vi "VELOCIDAD.vi"() -> ()   [LabVIEW 2023]
uses:
  <vilib>/Instr/_visa.llb/Select Event Type.ctl
  <vilib>/Instr/_visa.llb/VISA Configure Serial Port (Instr).vi
panel:
  out "Waveform Graph":dbl[](graph)
  out "Array":dbl[](array[numeric])
  in  "stop":bool
  in  "setpoint 2":dbl=1000.0
  in  "enviar":bool
  out "read buffer":string
  in  "Puerto":refnum<visa-resource-name>
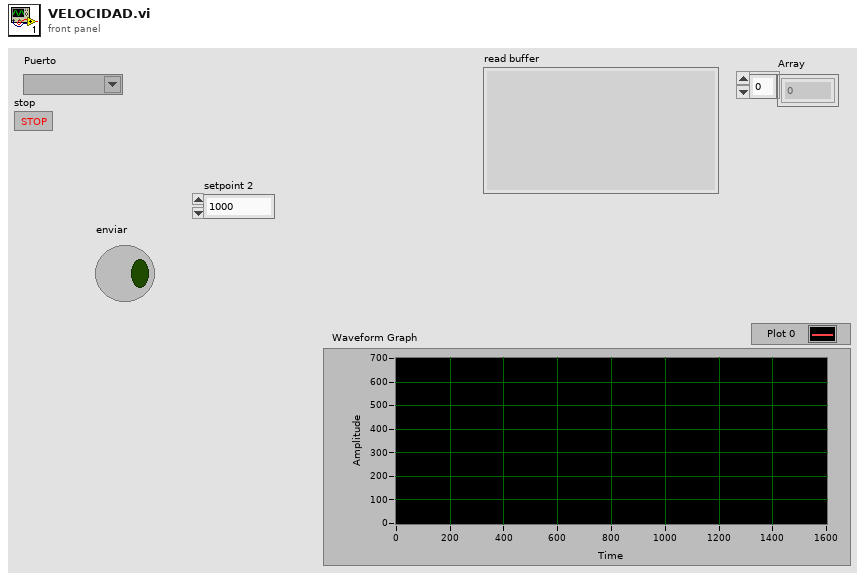
[diagram p1: front panel]
types:
  T1 = typedef "Select Event Type.ctl" = u32
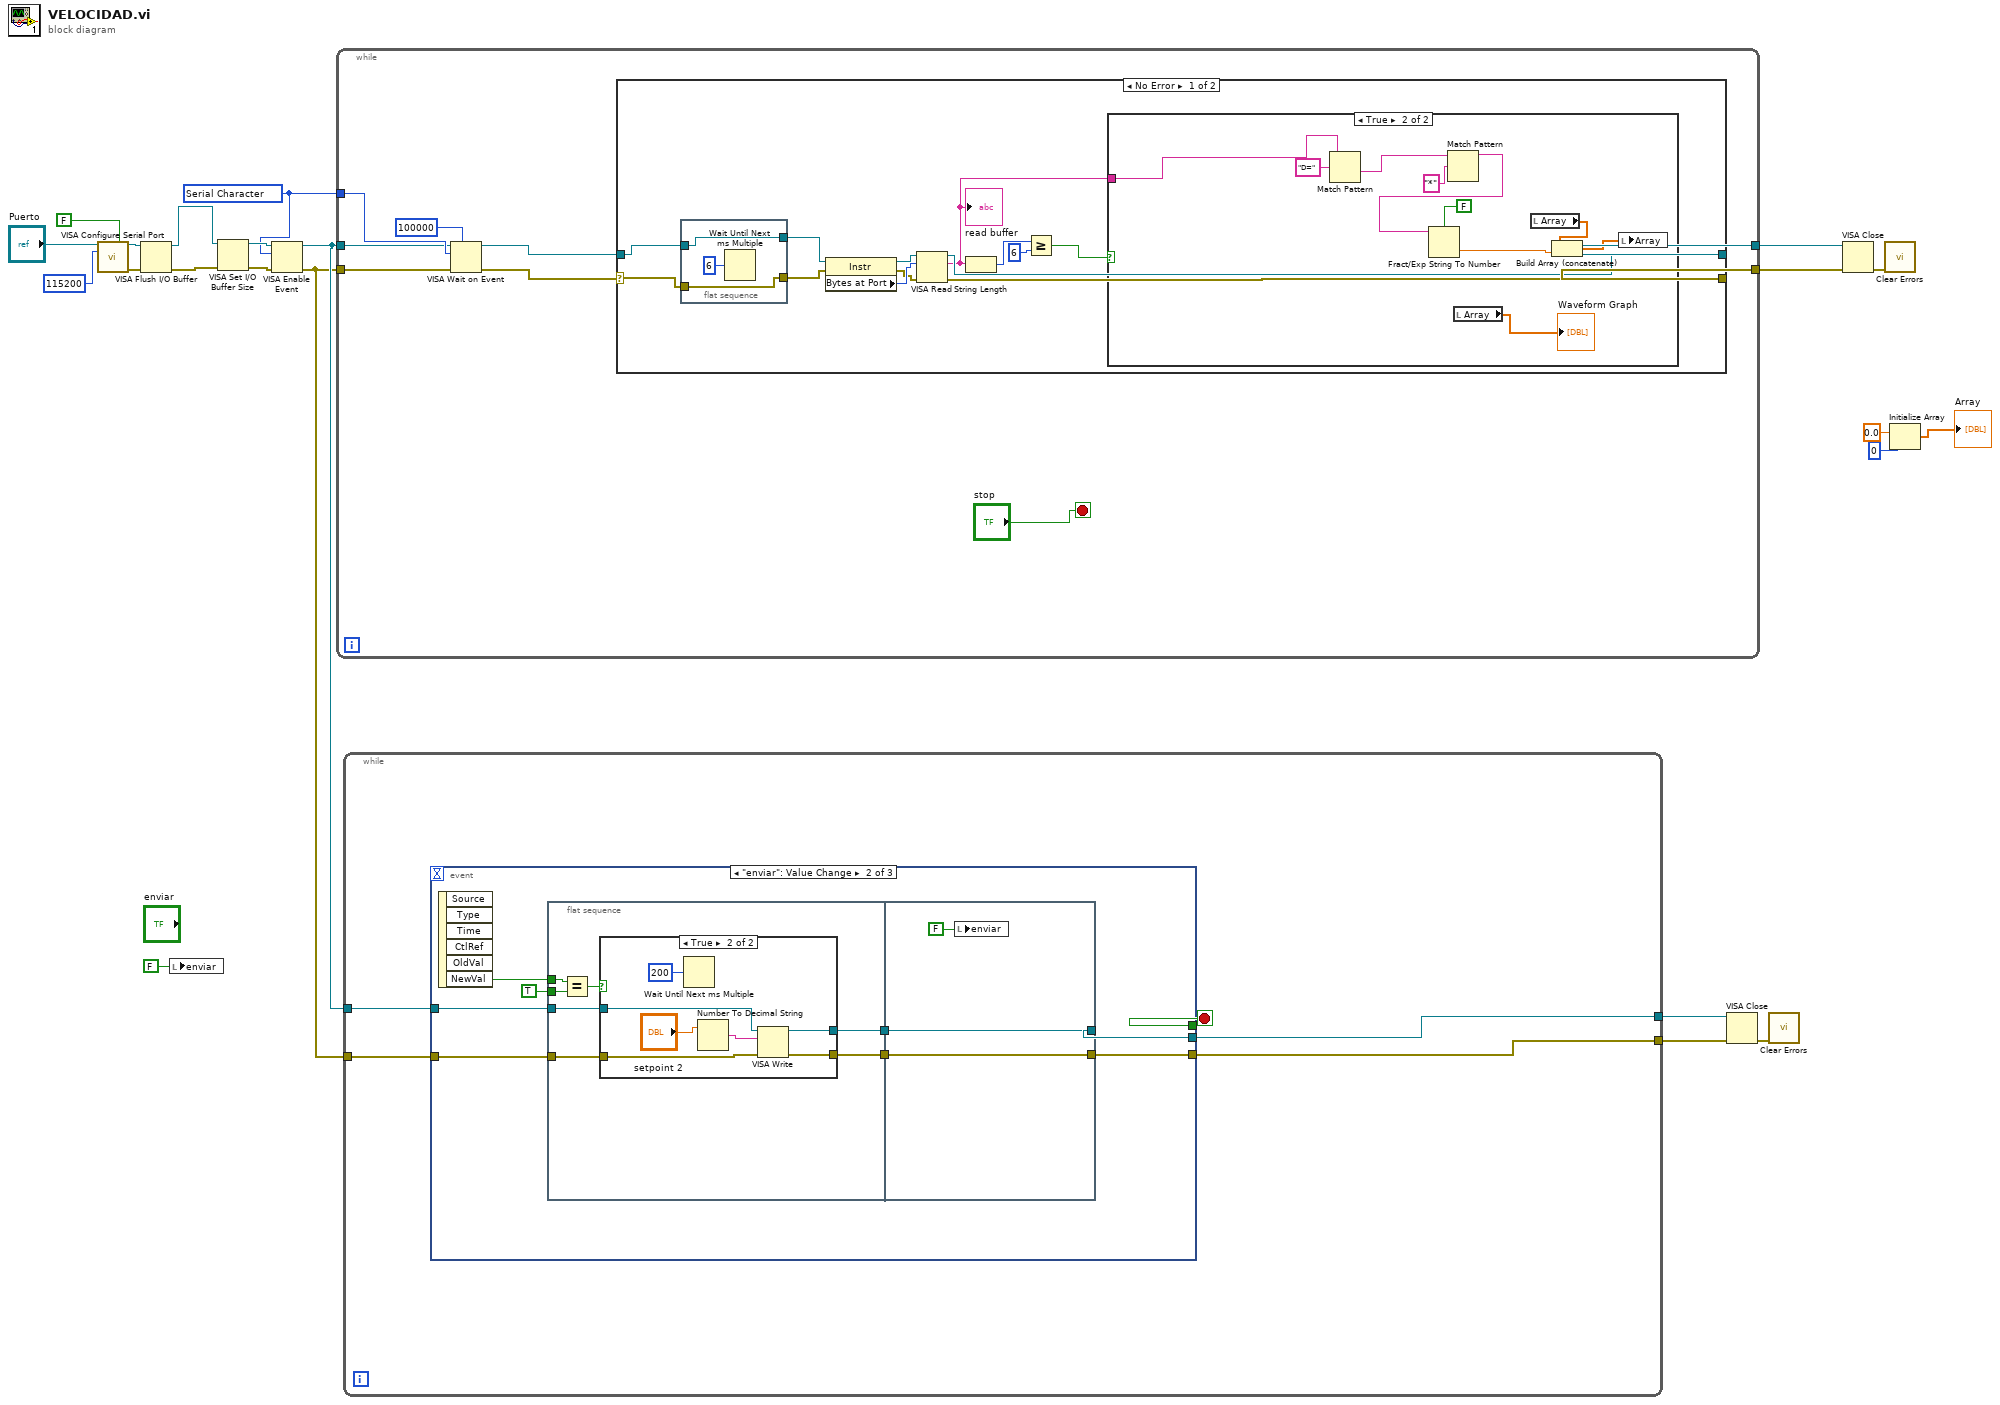
[diagram p0: block diagram]
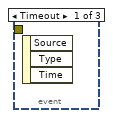
[diagram p2: hidden frame]
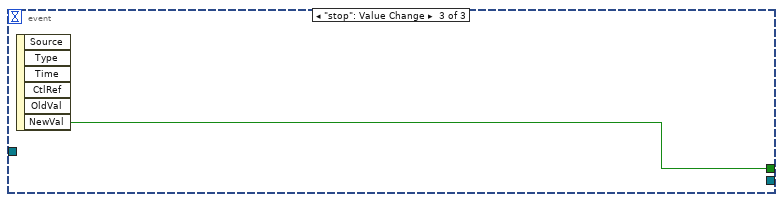
[diagram p4: hidden frame]
diagram:
  w13 = T1 1073684533 items=["Service Request"=1073684491, "Trigger"=3221168138, "Clear"=1073684493, "VXI Signal"=1073684512, "VXI/VME Interrupt"=3221168161, "VXI/VME Sysfail"=1073684509, "VXI/VME Sysreset"=1073684510, "GPIB CIC"=1073684498, "GPIB Talk"=1073684499, "GPIB Listen"=1073684500, "PXI Interrupt"=1073684514, "Serial Break"=1073684515, "Serial TermChar"=1073684516, "Serial CTS"=1073684521, "Serial DSR"=1073684522, "Serial DCD"=1073684524, "Serial RI"=1073684526, "Serial Character"=1073684533, "USB Interrupt"=1073684535, "All Enabled"=1073709055] ("Event Type")
  n1 = call-poly "VISA Configure Serial Port"("VISA resource name"="Puerto", "Enable Termination\nChar (T)"=FALSE ("Enable Termination\nChar (T)"), "baud rate (9600)"=u32 115200) -> ("VISA resource name out"=w19:refnum<visa-resource-name>, "error out"=w20:errorcluster)  [unwired: 11 in]
  n2 = VISA Flush I/O Buffer(VISA resource name=w19, error in (no error)=w20) -> (VISA resource name out=w17:refnum<visa-resource-name>, error out=w18:errorcluster)  [unwired: 1 in]
  n3 = local write "enviar"(FALSE ("enviar")) -> ()
  n4 = VISA Set I/O Buffer Size(VISA resource name=w17, error in (no error)=w18) -> (VISA resource name out=w15:refnum<visa-resource-name>, error out=w14:errorcluster)  [unwired: 2 in]
  n5 = VISA Enable Event ("VISA Enable \nEvent")(8:w14, 10:w13, 11:w15) -> (0:w4:errorcluster, 3:w5:refnum<visa-resource-name>)  [unwired: 1 out]
  n6 = while {
    tunnel: w5 -> [w25]
    tunnel: w4 -> [w24]
    tunnel: w13 -> [w31]
    tunnel: [w28] -> w12
    tunnel: [w27] -> w11
    stop <- "stop" stop-if-true
    n7 = VISA Wait on Event(7:u32 100000 ("timeout (0)"), 8:w24, 10:w31, 11:w25) -> (0:w29:errorcluster, 3:w30:refnum<visa-resource-name>)  [unwired: 3 out]
    n8 = case shown="No Error" w29 {
      selector: w29 -> [w35 w58]
      tunnel: w30 -> [w38 w59]
      tunnel: [w44 w58] -> w28
      tunnel: [w43 w59] -> w27
      frame No Error {
        n9 = flat-sequence {
          tunnel: w38 -> [w47]
          tunnel: [w47] -> w37
          tunnel: [w46] -> w36
          tunnel: w35 -> [w46]
          frame #0 {
            n10 = Wait Until Next ms Multiple(millisecond multiple=u32 6) -> ()  [unwired: 1 out]
          }
        }
        n11 = property class="Instr"(reference=w37, error in=w36) -> (reference out=w34:refnum<visa-resource-name>, error out=w32:errorcluster, "Bytes at Port"=w33:u32)
        n12 = VISA Read(VISA resource name=w34, byte count=w33, error in (no error)=w32) -> (VISA resource name out=w43:refnum<visa-resource-name>, read buffer=w39:string, error out=w44:errorcluster)  [unwired: 1 out]
        "read buffer" <- w39
        n13 = String Length(string=w39) -> (length=w42:i32)
        n14 = Greater Or Equal?(x=w42, y=6) -> (x >= y?=w40:bool)
        n15 = case shown="True" w40 {
          tunnel: w39 -> [_ w49]
          frame False {
          }
          frame True {
            n16 = Match Pattern(string=w49, regular expression="D=") -> (after substring=w55:string)  [unwired: 1 in, 3 out]
            n17 = Match Pattern(string=w55, regular expression="*") -> (before substring=w53:string)  [unwired: 1 in, 3 out]
            n18 = Fract/Exp String To Number(use system decimal point (T)=FALSE, string=w53) -> (number=w51:dbl)  [unwired: 2 in, 1 out]
            n19 = local read "Array"() -> (→"Waveform Graph":dbl[])
            n20 = local read "Array"() -> (w52:dbl[])
            n21 = Build Array (concatenate)(w52, w51) -> (w50:dbl[])
            n22 = local write "Array"(w50) -> ()
          }
        }
      }
      frame Error {
      }
    }
  }
  n23 = while {
    tunnel: [w64] -> w7
    tunnel: [w63] -> w6
    tunnel: w5 -> [w62]
    tunnel: w4 -> [w61]
    stop <- w60 stop-if-true
    n24 = event shown="[1] \"enviar\": Value Change" {
      selector: _ -> [_ _ _]
      dyn-events: _ -> [_ _ _]
      timeout: _ -> [_ _ _]
      tunnel: [_ w70 _] -> w64
      tunnel: [_ w69 _] -> w63
      tunnel: [_ _ w90] -> w60
      tunnel: w62 -> [_ w66 _]
      tunnel: w61 -> [_ w65 _]
      event Timeout {
        n25 = event-data() -> ()  [unwired: 1 in, 3 out]
      }
      event "enviar": Value Change {
        n26 = event-data() -> ("NewVal"=w72:bool)  [unwired: 1 in, 5 out]
        n27 = flat-sequence {
          tunnel: w72 -> [w79]
          tunnel: TRUE ("y") -> [w78]
          tunnel: [w76] -> w68
          tunnel: [w75] -> w67
          tunnel: w66 -> [w74]
          tunnel: w65 -> [w73]
          tunnel: [w88] -> w69
          tunnel: [w89] -> w70
          tunnel: w68 -> [w89]
          tunnel: w67 -> [w88]
          frame #0 {
            n28 = Equal?(x=w79, y=w78) -> (x = y?=w77:bool)
            n29 = case shown="True" w77 {
              tunnel: [_ w84] -> w76
              tunnel: [_ w83] -> w75
              tunnel: w74 -> [_ w81]
              tunnel: w73 -> [_ w80]
              frame False {
              }
              frame True {
                n30 = Wait Until Next ms Multiple(millisecond multiple=u32 200) -> ()  [unwired: 1 out]
                n31 = Number To Decimal String(number="setpoint 2") -> (decimal integer string=w85:string)  [unwired: 1 in]
                n32 = VISA Write(VISA resource name=w81, write buffer=w85, error in (no error)=w80) -> (VISA resource name out=w84:refnum<visa-resource-name>, error out=w83:errorcluster)  [unwired: 1 out]
              }
            }
          }
          frame #1 {
            n33 = local write "enviar"(FALSE ("enviar")) -> ()
          }
        }
      }
      event "stop": Value Change {
        n34 = event-data() -> ("NewVal"=w90:bool)  [unwired: 1 in, 5 out]
      }
    }
  }
  n35 = VISA Close(VISA resource name=w7, error in (no error)=w6) -> (error out=w9:errorcluster)
  n36 = call <vilib>:"Clear Errors.vi"("error in (no error)"=w9) -> ()  [unwired: 5 in, 2 out]
  n37 = VISA Close(VISA resource name=w11, error in (no error)=w12) -> (error out=w10:errorcluster)
  n38 = call <vilib>:"Clear Errors.vi"("error in (no error)"=w10) -> ()  [unwired: 5 in, 2 out]
  n39 = Initialize Array(0.0 ("element"), 0 ("dimension size")) -> (→"Array":dbl[])
